vi "Make Schema Details.vi"(4 "required?":bool, 5 "control itself?":bool, 6 "default value":variant, 7 "maximum":string, 8 "error in":errorcluster, 9 "minimum":string, 10 "unit note":string, 11 "description":string) -> (0 "error out":errorcluster, 3 "details":string)   [LabVIEW 2020, in "MCP Server.lvlib"]
doc: "Makes the JSON object of details that Add Control Details To Schema.vi merges into the schema of one control or element: description, minimum, maximum and default, each left out when there is none. The description is the element's description followed by the unit note. The control itself gets a description only when it has a unit note, and a default only when it is not required (left out above 1024 characters). Elements never get a default."
uses:
  MCP Server.lvlib
  d13a1dd9-aee2-4240-a612-40fb2030387e.vi
  e705c3ca-6da0-4e96-b22a-f352743e0055.vi
  <vilib>/JDP Science/JSONtext/Variant to JSON Text.vi
  <vilib>/JDP Science/JSONtext/support/Format JSON Object.vi
  <vilib>/JDP Science/JSONtext/LVClass Serializer/JSONtext LVClass Serializer.lvclass
  <vilib>/JDP Science/JSONtext/JSONtext.lvlib
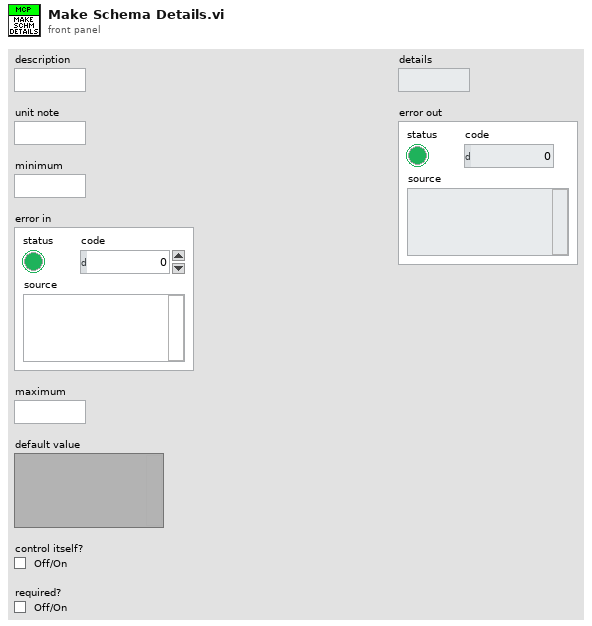
[diagram p1: front panel]
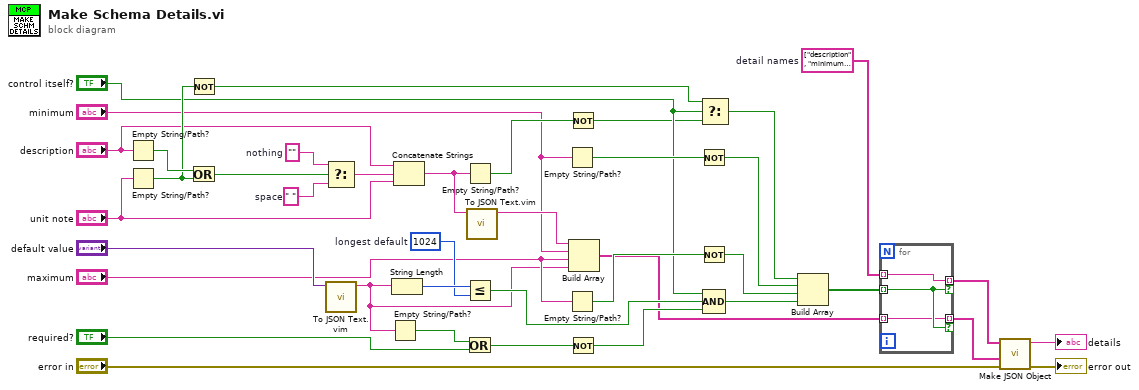
[diagram p0: block diagram]
diagram:
  w8 = string[] ["description", "minimum", "maximum", "default"]  # detail names
  w37 = 1024  # longest default
  w27 = ""  # nothing
  w25 = " "  # space
  n1 = Empty String/Path?(string/path="description") -> (empty?=w29:bool)
  n2 = Empty String/Path?(string/path="unit note") -> (empty?=w28:bool)
  n3 = Not(x=w28) -> (.not. x?=w19:bool)
  n4 = Or(x=w29, y=w28) -> (x .or. y?=w26:bool)
  n5 = Select(t=w27, s=w26, f=w25) -> (s? t:f=w23:string)
  n6 = call "To JSON Text.vim"("Anything"="default value") -> ("<JSON>"=w13:string)  [unwired: 9 in, 1 out]
  n7 = Empty String/Path?(string/path=w13) -> (empty?=w36:bool)
  n8 = String Length(string=w13) -> (length=w38:i32)
  n9 = Concatenate Strings("description", w23, "unit note") -> (w21:string)
  n10 = Empty String/Path?(string/path=w21) -> (empty?=w20:bool)
  n11 = Less Or Equal?(x=w38, y=w37) -> (x <= y?=w33:bool)
  n12 = Or(x=w36, y="required?") -> (x .or. y?=w34:bool)
  n13 = call "To JSON Text.vim"("Anything"=w21) -> ("<JSON>"=w16:string)  [unwired: 9 in, 1 out]
  n14 = Empty String/Path?(string/path="minimum") -> (empty?=w31:bool)
  n15 = Empty String/Path?(string/path="maximum") -> (empty?=w30:bool)
  n16 = Not(x=w20) -> (.not. x?=w17:bool)
  n17 = Not(x=w34) -> (.not. x?=w32:bool)
  n18 = Build Array(w16, "minimum", "maximum", w13) -> (w7:string[])
  n19 = Not(x=w31) -> (.not. x?=w11:bool)
  n20 = Not(x=w30) -> (.not. x?=w10:bool)
  n21 = Select(t=w19, s="control itself?", f=w17) -> (s? t:f=w12:bool)
  n22 = Compound Arithmetic op=AND("control itself?", w33, w32) -> (w9:bool)
  n23 = Build Array(w12, w11, w10, w9) -> (w6:bool[])
  n24 = for {
    tunnel: w8 -> [w42] mode=indexing
    tunnel: w7 -> [w40] mode=indexing
    tunnel: w6 -> [w41] mode=indexing
    tunnel: [w42] -> w5 mode=indexing if=w41
    tunnel: [w40] -> w4 mode=indexing if=w41
  }
  n25 = call <vilib>:"Make JSON Object.vi"("error in (no error)"="error in", "JSON Items"=w4, "Item Names"=w5) -> ("error out"=→"error out":errorcluster, "<JSON>"=→"details":string)  [unwired: 7 in]
